vi "Load Config.vi"(8 "error in (no error)":errorcluster, 11 "GUI Manager Module in":refnum<class "GUI Manager Module.lvclass">) -> (0 "error out":errorcluster, 3 "GUI Manager Module out":refnum<class "GUI Manager Module.lvclass">)   [LabVIEW 2020, in "VolatusGUI.lvlib" / "GUI Manager Module.lvclass"]
uses:
  GUI Manager Module.lvclass
  C:/dev/lv20CE/relink/lv-volatus/Volatus/Module/Module.lvclass
  Volatus/Module/Module.lvclass/Module.ctl
  VolatusConfig/VolatusConfigElement/VolatusConfigElement.lvclass/VolatusConfigElement.ctl
  GUI Manager Module.lvclass/GUI Manager Module.ctl
  Volatus/Module/Config.vi
  VolatusConfig/VolatusConfigElement/Element.vi
  VolatusConfig/Task/Task Config.lvclass
  C:/dev/lv20CE/relink/lv-volatus/VolatusConfig/VolatusConfigElement/VolatusConfigElement.lvclass
  Volatus/Module/Module.lvclass
  VolatusConfig/VolatusConfigElement/VolatusConfigElement.lvclass
  lv-cdm/CDM-Config/Config Element/Config Element.lvclass
  C:/dev/lv20CE/relink/lv-volatus/VolatusGUI/GUI Manager Module/GUI Manager Module.lvclass
  C:/dev/lv20CE/relink/lv-volatus/VolatusConfig/Task/Task Config.lvclass
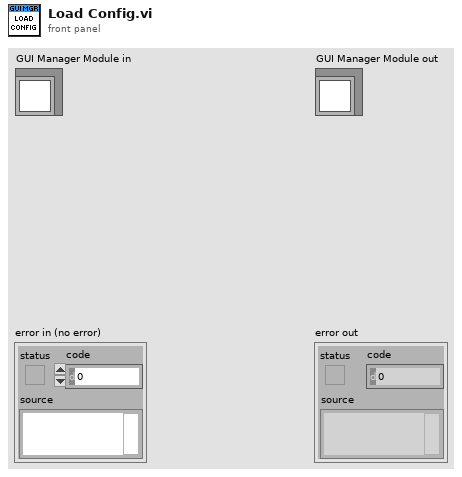
[diagram p1: front panel]
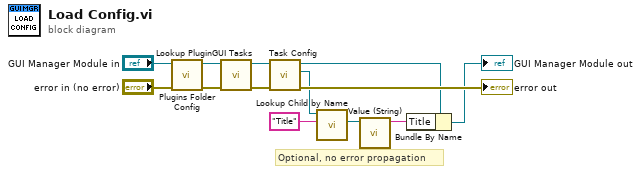
[diagram p0: block diagram]
diagram:
  # "Optional, no error propagation"
  n1 = call "Plugins Folder Config.vi"("error in (no error)"="error in (no error)", "GUI Manager Module in"="GUI Manager Module in") -> ("error out"=w10:errorcluster, "GUI Manager Module out"=w11:refnum<class "GUI Manager Module.lvclass">)  [unwired: 8 in]
  n2 = call "Lookup PluginGUI Tasks.vi"("error in (no error)"=w10, "GUI Manager Module in"=w11) -> ("error out"=w9:errorcluster, "GUI Manager Module out"=w7:refnum<class "GUI Manager Module.lvclass">)  [unwired: 8 in]
  n3 = call "Task Config.vi"("error in (no error)"=w9, "Module in"=w7) -> ("error out"=→"error out":errorcluster, "Task Config"=w5:refnum<class "Task Config.lvclass">, "Module out"=w6:refnum<class "GUI Manager Module.lvclass">)  [unwired: 7 in]
  n4 = call "Lookup Child by Name.vi"("Child Name"="Title", "VolatusConfigElement in"=w5) -> ("Child"=w2:refnum<class "Config Element.lvclass">)  [unwired: 6 in, 3 out]
  n5 = call "Value (String).vi"("Config Element in"=w2) -> ("String Value"=w1:string)  [unwired: 9 in, 1 out]
  n6 = Bundle By Name(cluster=w6, "Title"=w1) -> (→"GUI Manager Module out":refnum<class "GUI Manager Module.lvclass">)
